vi "TrajectoryParam_enforceAccel.vi"(8 "TRAJECTORY_CONFIG":T1 {"End Velocity" format="%20.4f"; "StartVelocity" format="%20.4f"; "Max Acceleration" format="%20.4f"; "MaxVelocity" format="%20.4f"}, 10 "Reversed":bool, 11 "inCONSTRAINED_STATE":T2={"POSEwCURVATURE"={"CURVATURE"=0.0, "POSE"={"TRANSLATION"={"X"=0.0, "Y"=0.0}, "ROTATION"={"VALUE"=0.0, "COS"=1.0, "SIN"=0.0}}}, "Distance"=0.0, "minAccel"=0.0, "maxAccel"=0.0, "maxVelocity"=0.0} {"POSEwCURVATURE"."POSE"."ROTATION"."SIN" format="%13.4f"; "POSEwCURVATURE"."POSE"."ROTATION"."COS" format="%13.4f"; "POSEwCURVATURE"."POSE"."ROTATION"."VALUE" format="%13.4f"; "POSEwCURVATURE"."POSE"."TRANSLATION"."Y" format="%14.3f"; "POSEwCURVATURE"."POSE"."TRANSLATION"."X" format="%14.3f"}) -> (0 "error out":errorcluster, 3 "outCONSTRAINED_STATE":T2={"POSEwCURVATURE"={"CURVATURE"=0.0, "POSE"={"TRANSLATION"={"X"=0.0, "Y"=0.0}, "ROTATION"={"VALUE"=0.0, "COS"=1.0, "SIN"=0.0}}}, "Distance"=0.0, "minAccel"=0.0, "maxAccel"=0.0, "maxVelocity"=0.0} {"POSEwCURVATURE"."POSE"."ROTATION"."SIN" format="%13.4f"; "POSEwCURVATURE"."POSE"."ROTATION"."COS" format="%13.4f"; "POSEwCURVATURE"."POSE"."ROTATION"."VALUE" format="%13.4f"; "POSEwCURVATURE"."POSE"."TRANSLATION"."Y" format="%14.3f"; "POSEwCURVATURE"."POSE"."TRANSLATION"."X" format="%14.3f"})   [LabVIEW 2019, in "Trajectory_Library.lvlib"]
doc: "Internal routine called by TrajectoryParam_timeParam.VI \n\nThis routine enforces acceleration constraints and updates the ConstrainedState value based on the calculated limits.\n\nThis routine will need to be updated whenever a new constrained state type is added.\n------------------------------------------------------------------------------------------\n\nParameters:\n - InConstrainedState\n - Reversed\n - TrajectoryConfig\n\nReturns\n - OutConstrainedState"
uses:
  Trajectory_Library.lvlib
  <vilib>/Utility/Data Type/NI_Data Type.lvlib
  TypeDef/TRAJ_CONSTRAINT_CENTRIPETAL_ACCEL.ctl
  TypeDef/DIFF_DRIVE_KINEMATICS.ctl
  TypeDef/TRAJ_CONSTRAINT_DIIF_DRIVE_KINEMATICS.ctl
  TypeDef/SIMPLE_MOTOR_FF.ctl
  TypeDef/TRAJ_CONSTRAINT_DIIF_DRIVE_VOLTAGE.ctl
  TypeDef/TRANSLATION2D.ctl
  <vilib>/Analysis/Matrix/Datatypes/RealMatrix.ctl
  <vilib>/Analysis/Matrix/NI_Matrix.lvlib
  TypeDef/MECA_DRIVE_KINEMATICS.ctl
  TypeDef/TRAJ_CONSTRAINT_MECA_DRIVE_KINEMATICS.ctl
  TypeDef/SWERVE_DRIVE_KINEMATICS.ctl
  TypeDef/TRAJ_CONSTRAINT_SWERVE_DRIVE_KINEMATICS.ctl
  TypeDef/TRAJ_CONSTRAINT_MAX_VELOCITY.ctl
  Enum/TRAJ_CONSTRAINT_TYPES_ENUM.ctl
  TypeDef/TRAJ_CONSTRAINT_ELLIP_REGION.ctl
  TypeDef/TRAJ_CONSTRAINT_RECT_REGION.ctl
  TypeDef/ROTATION2D.ctl
  TypeDef/SWERVE_DRIVE_MODULE_STATE.ctl
  TypeDef/POSE2D.ctl
  TypeDef/POSEwCURVATURE.ctl
  TypeDef/CONSTRAINED_STATE.ctl
  TypeDef/TRAJ_CONFIG.ctl
panel:
  # "All units\nare SI"
  # "All units\nare SI"
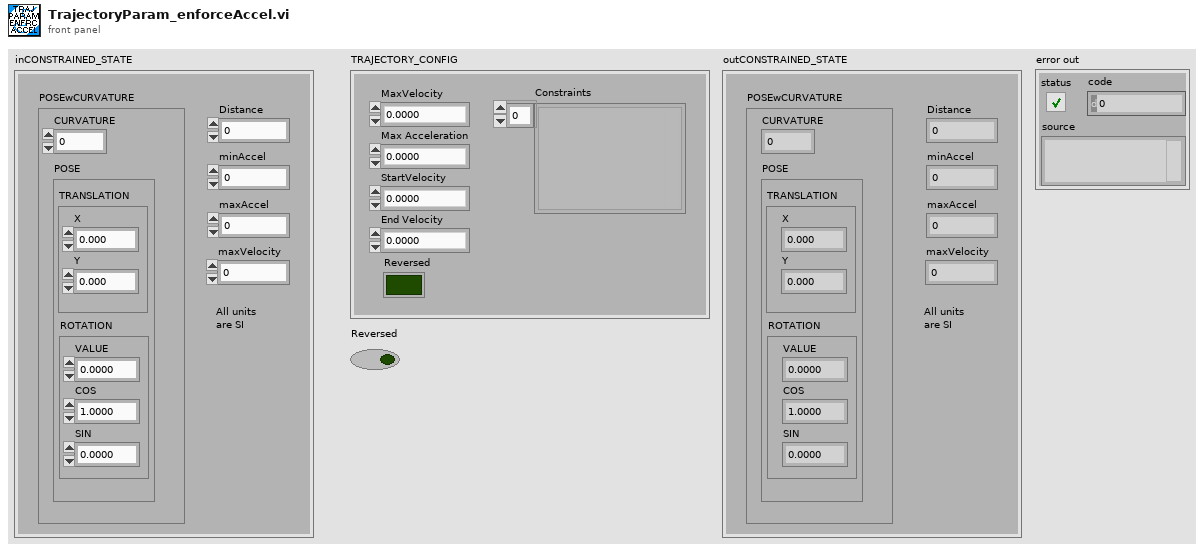
[diagram p1: front panel]
types:
  T1 = typedef "Trajectory_Library.lvlib/TRAJ_CONFIG.ctl" = cluster{"MaxVelocity":dbl, "Max Acceleration":dbl, "StartVelocity":dbl, "End Velocity":dbl, "Reversed":bool, "Constraints":variant[]}
  T2 = typedef "Trajectory_Library.lvlib/CONSTRAINED_STATE.ctl" = cluster{"POSEwCURVATURE":T3, "Distance":dbl, "minAccel":dbl, "maxAccel":dbl, "maxVelocity":dbl}
  T3 = typedef "Trajectory_Library.lvlib/POSEwCURVATURE.ctl" = cluster{"CURVATURE":dbl, "POSE":T4}
  T4 = typedef "Trajectory_Library.lvlib/POSE2D.ctl" = cluster{"TRANSLATION":T5, "ROTATION":T6}
  T5 = typedef "Trajectory_Library.lvlib/TRANSLATION2D.ctl" = cluster{"X":dbl, "Y":dbl}
  T6 = typedef "Trajectory_Library.lvlib/ROTATION2D.ctl" = cluster{"VALUE":dbl, "COS":dbl, "SIN":dbl}
  T7 = typedef "Trajectory_Library.lvlib/TRAJ_CONSTRAINT_DIIF_DRIVE_KINEMATICS.ctl" = cluster{"Max Speed (M/S)":dbl, "DIFF_DRIVE_KINEMATICS":T8, "Max Accel (M/S2)":dbl}
  T8 = typedef "Trajectory_Library.lvlib/DIFF_DRIVE_KINEMATICS.ctl" = cluster{"TrackWidth_Meters":dbl}
  T9 = typedef "Trajectory_Library.lvlib/TRAJ_CONSTRAINT_CENTRIPETAL_ACCEL.ctl" = cluster{"Max Cent Accel":dbl}
  T10 = typedef "Trajectory_Library.lvlib/TRAJ_CONSTRAINT_DIIF_DRIVE_VOLTAGE.ctl" = cluster{"Max Voltage":dbl, "DIFF_DRIVE_KINEMATICS":T8, "SIMPLE_MOTOR_FF":T11}
  T11 = typedef "Trajectory_Library.lvlib/SIMPLE_MOTOR_FF.ctl" = cluster{"Ks":dbl, "Kv":dbl, "Ka":dbl, "KnInv":dbl}
  T12 = typedef "Trajectory_Library.lvlib/TRAJ_CONSTRAINT_MECA_DRIVE_KINEMATICS.ctl" = cluster{"Max Speed (M/S)":dbl, "MECA_DRIVE_KINEMATICS":T13}
  T13 = typedef "Trajectory_Library.lvlib/MECA_DRIVE_KINEMATICS.ctl" = cluster{"FrontLeft":T5, "FrontRight":T5, "RearLeft":T5, "RearRight":T5, "InverseKinematics":T14, "ForwardKinematics":T14, "PrevCoR":T5}
  T14 = typedef "NI_Matrix.lvlib/RealMatrix.ctl" = dbl[][]
  T15 = typedef "Trajectory_Library.lvlib/TRAJ_CONSTRAINT_SWERVE_DRIVE_KINEMATICS.ctl" = cluster{"Max Speed (M/S)":dbl, "SwerveKinematics":T16}
  T16 = typedef "Trajectory_Library.lvlib/SWERVE_DRIVE_KINEMATICS.ctl" = cluster{"NumModules":i32, "InverseKinematics":T14, "ForwardKinematics":T14, "Modules":T5[], "PrevCoR":T5, "SavedModuleStates":T17[]}
  T17 = typedef "Trajectory_Library.lvlib/SWERVE_DRIVE_MODULE_STATE.ctl" = cluster{"Speed":dbl, "Angle":T6}
  T18 = typedef "Trajectory_Library.lvlib/TRAJ_CONSTRAINT_MAX_VELOCITY.ctl" = cluster{"Max Velocity":dbl, "IM UNIQUE":bool}
  T19 = typedef "Trajectory_Library.lvlib/TRAJ_CONSTRAINT_ELLIP_REGION.ctl" = cluster{"Center":T5, "Radii":T5, "Constraint":variant, "Constraint Type":T20, "IM UNIQUE":bool}
  T20 = typedef "Trajectory_Library.lvlib/TRAJ_CONSTRAINT_TYPES_ENUM.ctl" = enum16{"UNDEFINED", "DIFF DRIVE KINEMATICS", "DIFF DRIVE VOLTAGE", "CENTRIPITAL ACCEL", "MECA DRIVE KINEMATICS", "SWERVE DRIVE KINEMATICS", "MAXIMUM VELOCITY", "ELLIPTICAL REGION", "RECTANGULAR REGION"}
  T21 = typedef "Trajectory_Library.lvlib/TRAJ_CONSTRAINT_RECT_REGION.ctl" = cluster{"BottomLeftPoint":T5, "TopRightPoint":T5, "Constraint":variant, "Constraint Type":T20}
  T22 = typedef "Trajectory_Library.lvlib/TRAJ_CONSTRAINT_MINMAX.ctl" = cluster{"minAccel":dbl, "maxAccel":dbl}
  T23 = typedef "WPILib_Math.lvlib/TRAJ_CONSTRAINT_MINMAX.ctl" = cluster{"minAccel":dbl, "maxAccel":dbl}
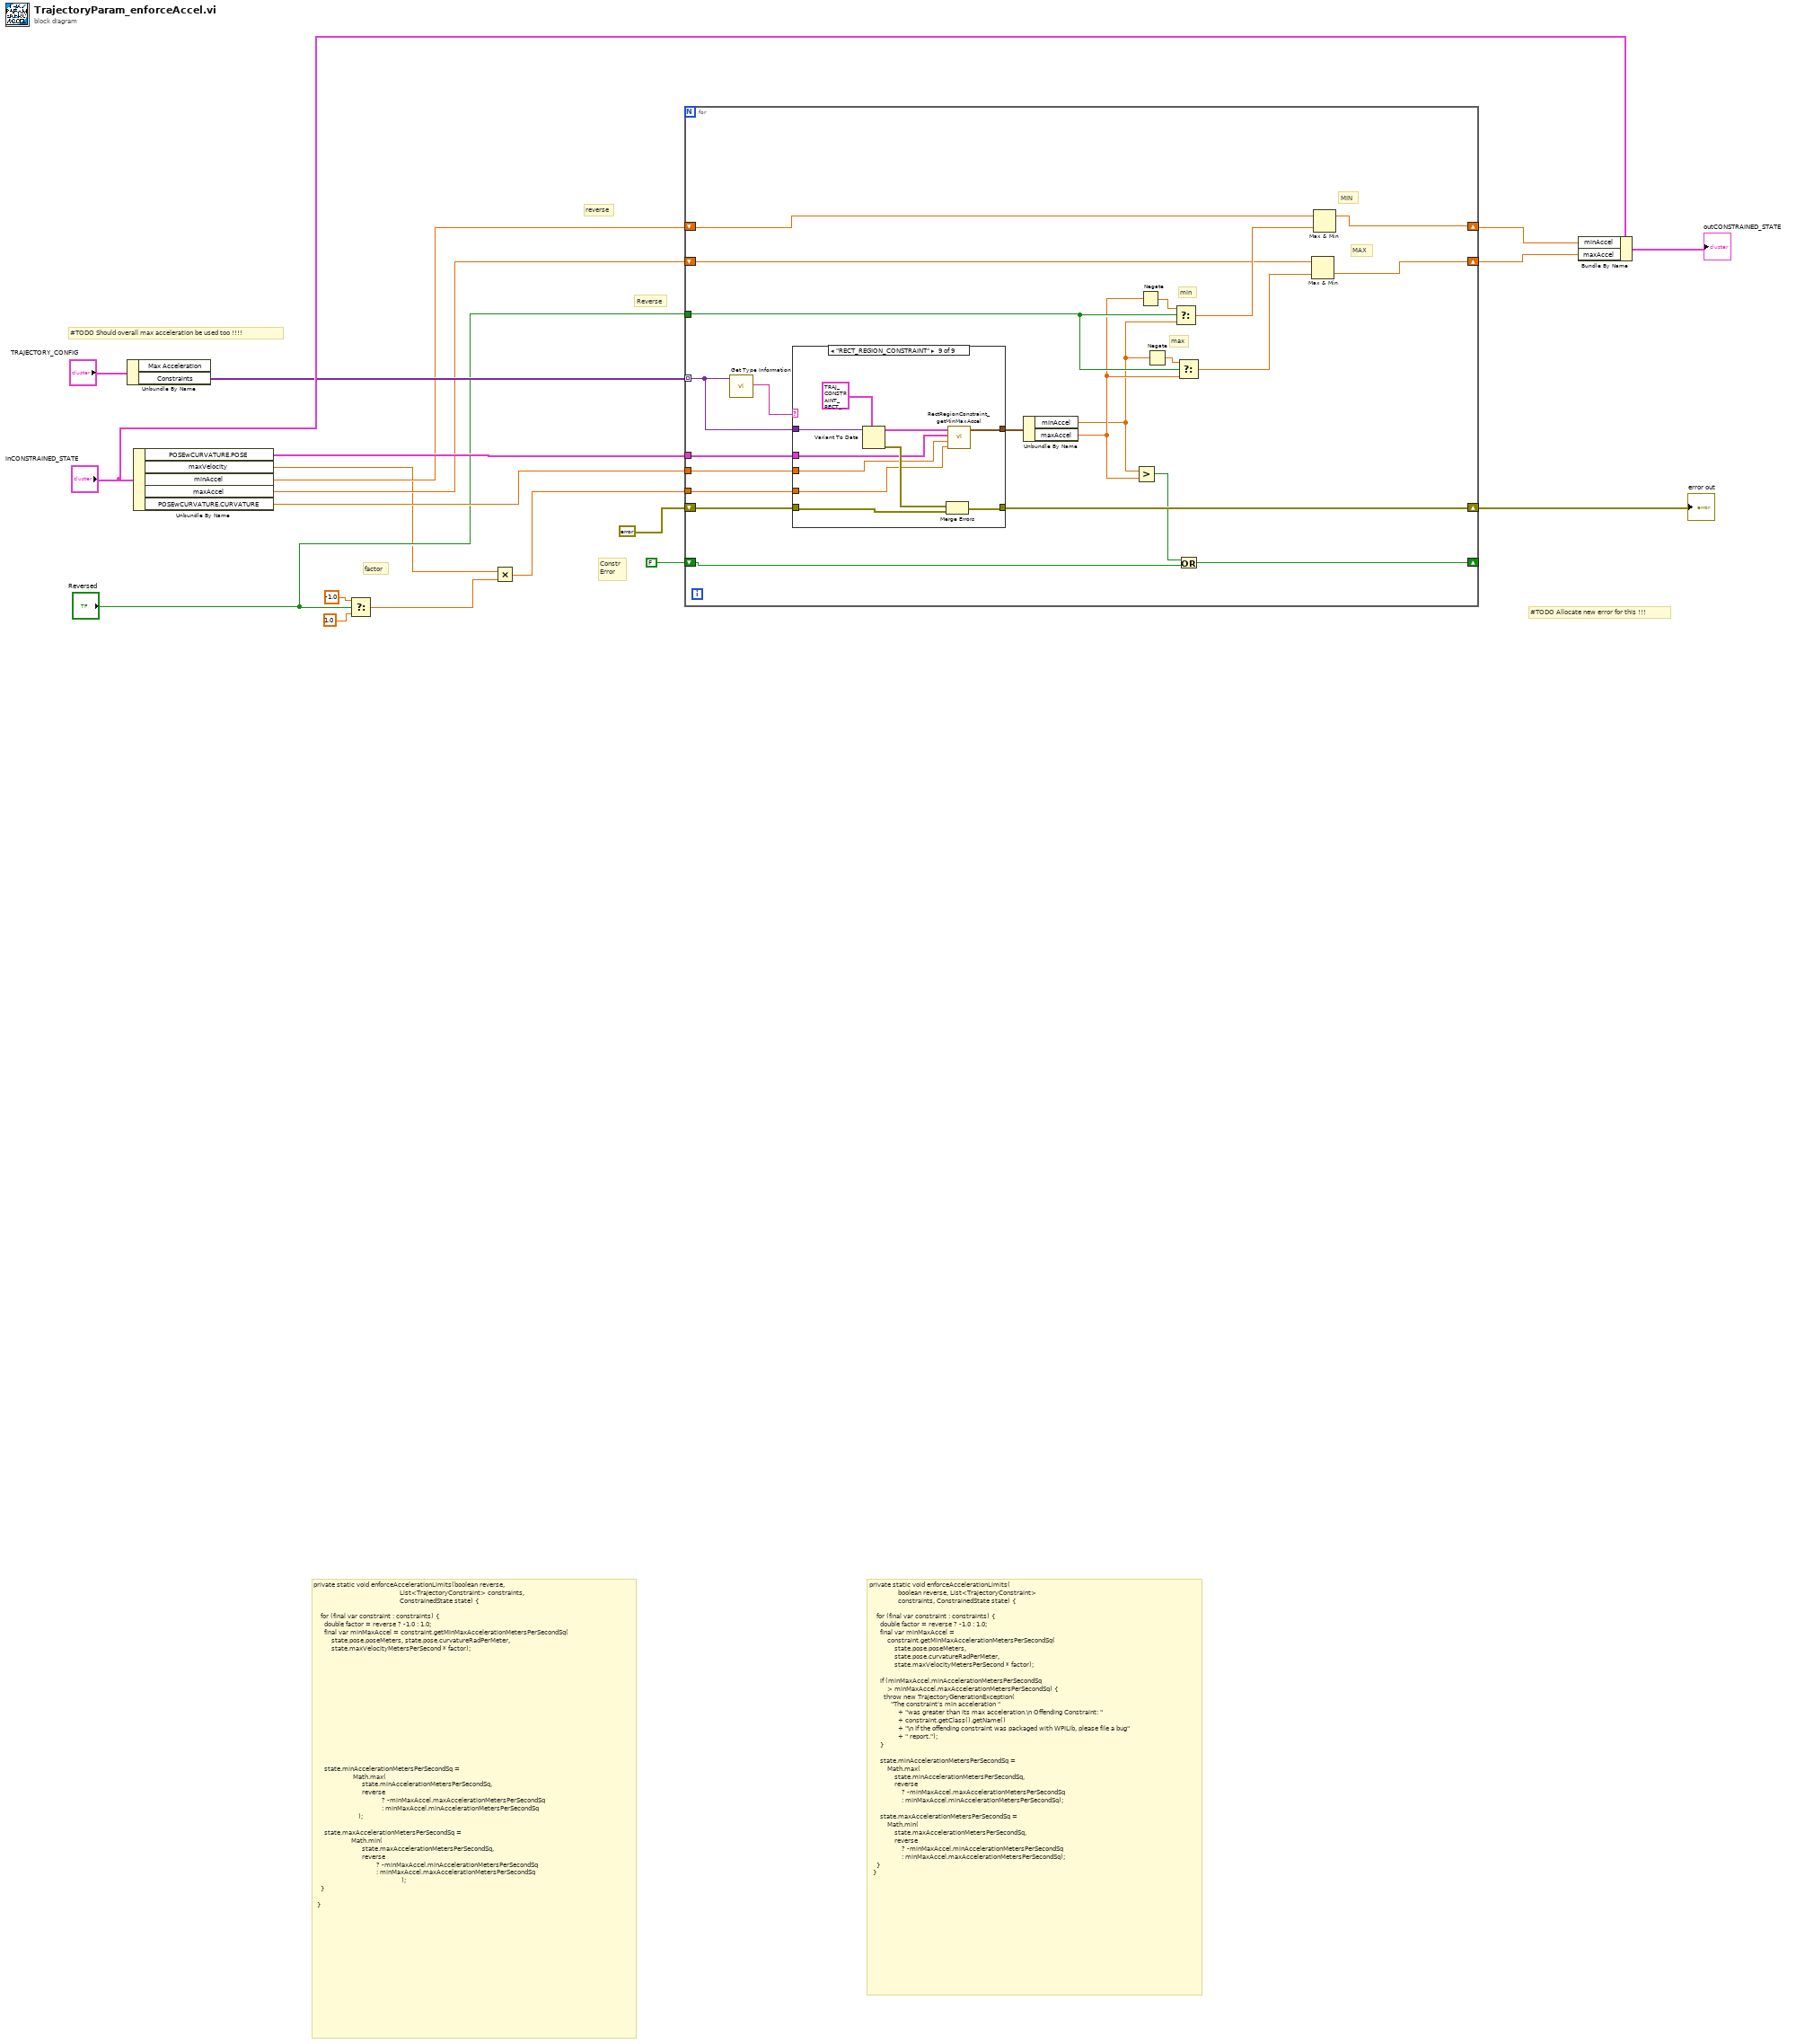
[diagram p0: block diagram]
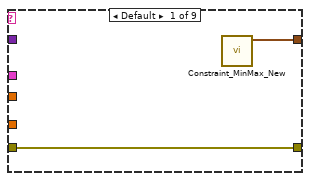
[diagram p2: hidden frame]
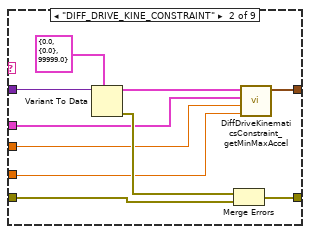
[diagram p3: hidden frame]
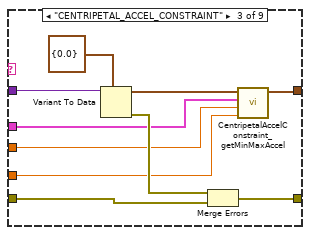
[diagram p4: hidden frame]
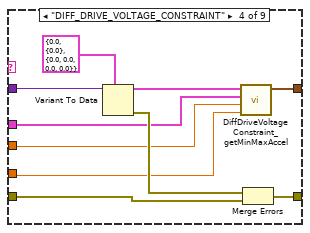
[diagram p5: hidden frame]
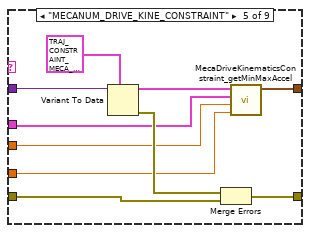
[diagram p6: hidden frame]
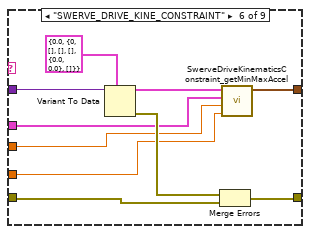
[diagram p7: hidden frame]
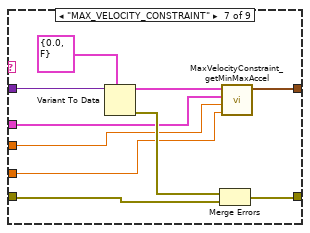
[diagram p8: hidden frame]
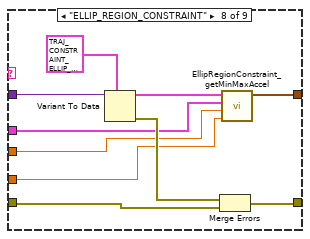
[diagram p9: hidden frame]
diagram:
  # "#TODO Allocate new error for this !!!"
  # "#TODO Should overall max acceleration be used too !!!!"
  # "Reverse"
  # "reverse"
  # "Constr\nError"
  # "private static void enforceAccelerationLimits(\n                boolean reverse, List<TrajectoryConstraint> \n                constraints, ConstrainedState state) {\n\n    for (final var constraint : constraints) {\n      double factor = reverse ? -1.0 : 1.0;\n      final var minMaxAccel =\n          constraint.getMinMaxAccelerationMetersPerSecondSq(\n              state.pose.poseMeters,\n              state.pose.curvatureRadPerMeter,\n              state.maxVelocityMetersPerSecond * factor);\n\n      if (minMaxAccel.minAccelerationMetersPerSecondSq\n          > minMaxAccel.maxAccelerationMetersPerSecondSq) {\n        throw new TrajectoryGenerationException(\n            \"The constraint's min acceleration \"\n                + \"was greater than its max acceleration.\\n Offending Constraint: \"\n                + constraint.getClass().getName()\n                + \"\\n If the offending constraint was packaged with WPILib, please file a bug\"\n                + \" report.\");\n      }\n\n      state.minAccelerationMetersPerSecondSq =\n          Math.max(\n              state.minAccelerationMetersPerSecondSq,\n              reverse\n                  ? -minMaxAccel.maxAccelerationMetersPerSecondSq\n                  : minMaxAccel.minAccelerationMetersPerSecondSq);\n\n      state.maxAccelerationMetersPerSecondSq =\n          Math.min(\n              state.maxAccelerationMetersPerSecondSq,\n              reverse\n                  ? -minMaxAccel.minAccelerationMetersPerSecondSq\n                  : minMaxAccel.maxAccelerationMetersPerSecondSq);\n    }\n  }"
  # "factor"
  # "private static void enforceAccelerationLimits(boolean reverse,\n                                                List<TrajectoryConstraint> constraints,\n                                                ConstrainedState state) {\n\n    for (final var constraint : constraints) {\n      double factor = reverse ? -1.0 : 1.0;\n      final var minMaxAccel = constraint.getMinMaxAccelerationMetersPerSecondSq(\n          state.pose.poseMeters, state.pose.curvatureRadPerMeter,\n          state.maxVelocityMetersPerSecond * factor);\n\n\n\n\n\n\n\n\n\n\n\n\n\n\n      state.minAccelerationMetersPerSecondSq = \n                      Math.max(\n                           state.minAccelerationMetersPerSecondSq,\n                           reverse \n                                      ? -minMaxAccel.maxAccelerationMetersPerSecondSq \n                                      : minMaxAccel.minAccelerationMetersPerSecondSq\n                         );\n\n      state.maxAccelerationMetersPerSecondSq = \n                     Math.min(\n                           state.maxAccelerationMetersPerSecondSq,\n                           reverse \n                                   ? -minMaxAccel.minAccelerationMetersPerSecondSq \n                                   : minMaxAccel.maxAccelerationMetersPerSecondSq\n                                                 );\n    }\n\n  }"
  n1 = Unbundle By Name("TRAJECTORY_CONFIG") -> ("Constraints"=w14:variant[])  [unwired: 1 out]
  n2 = Unbundle By Name("inCONSTRAINED_STATE") -> ("POSEwCURVATURE.POSE"=w12:T4, "maxVelocity"=w2:dbl, "minAccel"=w6:dbl, "maxAccel"=w7:dbl, "POSEwCURVATURE.CURVATURE"=w11:dbl)
  n3 = Select(t=-1.0, s="Reversed", f=1.0) -> (s? t:f=w1:dbl)
  n4 = Multiply(x=w2, y=w1) -> (x*y=w10:dbl)
  n5 = for {
    tunnel: w14 -> [w40] mode=indexing
    tunnel: w12 -> [w39]
    tunnel: w11 -> [w38]
    tunnel: w10 -> [w37]
    shift-right: [w36] -> w5
    shift-left: errorcluster {"status"=FALSE, "code"=0, "source"=""} ("error IO") -> [w35]
    shift-right: [w32] -> _
    shift-left: FALSE -> [w31]
    tunnel: "Reversed" -> [w30]
    shift-right: [w22] -> w4
    shift-left: w6 -> [w27]
    shift-right: [w21] -> w3
    shift-left: w7 -> [w25]
    # "MAX"
    # "MIN"
    # "max"
    # "min"
    n6 = call <vilib>:"Get Type Information.vi"("variant"=w40) -> ("name"=w41:string)  [unwired: 6 in, 4 out]
    n7 = case shown="\"RECT_REGION_CONSTRAINT\"" w41 {
      tunnel: w40 -> [_ w53 w63 w73 w83 w93 w103 w113 w123]
      tunnel: w39 -> [_ w46 w56 w66 w76 w87 w97 w107 w117]
      tunnel: w38 -> [_ w45 w55 w65 w75 w86 w96 w106 w116]
      tunnel: w37 -> [_ w44 w54 w64 w74 w85 w95 w105 w115]
      tunnel: [w43 w51 w62 w71 w82 w92 w102 w112 w122] -> w36
      tunnel: w35 -> [w43 w50 w60 w70 w80 w90 w100 w110 w120]
      tunnel: [w42 w48 w58 w68 w78 w84 w94 w104 w114] -> w34
      frame Default {
        n8 = call "Constraint_MinMax_New.vi"() -> ("TRAJ_CONSTAINT_MIN_MAX"=w42:T22)  [unwired: 11 in]
      }
      frame "DIFF_DRIVE_KINE_CONSTRAINT" {
        n9 = Variant To Data(type=T7 {"Max Speed (M/S)"=0.0, "DIFF_DRIVE_KINEMATICS"={"TrackWidth_Meters"=0.0}, "Max Accel (M/S2)"=99999.0} ("DIFF_DRIVE_KINE_CONSTRAINT"), Variant=w53) -> (data=w47:T7, error out=w52:errorcluster)  [unwired: 1 in]
        n10 = Merge Errors(w52, w50) -> (w51:errorcluster)
        n11 = call "DiffDriveKinematicsConstraint_getMinMaxAccel.vi"("Velocity_M/S"=w44, "Curvature"=w45, "statePose"=w46, "DIFF_DRIVE_KINE_CONSTRAINT"=w47) -> ("TRAJ_CONSTAINT_MIN_MAX"=w48:T23)  [unwired: 7 in]
      }
      frame "CENTRIPETAL_ACCEL_CONSTRAINT" {
        n12 = Variant To Data(type=T9 {"Max Cent Accel"=0.0} ("CENTRIPETAL_ACCEL_CONSTRAINT"), Variant=w63) -> (data=w57:T9, error out=w61:errorcluster)  [unwired: 1 in]
        n13 = Merge Errors(w61, w60) -> (w62:errorcluster)
        n14 = call "CentripetalAccelConstraint_getMinMaxAccel.vi"("maxVelocity"=w54, "Curvature"=w55, "statePose"=w56, "CENTRIPETAL_ACCEL_CONSTRAINT"=w57) -> ("TRAJ_CONSTAINT_MIN_MAX"=w58:T23)  [unwired: 7 in]
      }
      frame "DIFF_DRIVE_VOLTAGE_CONSTRAINT" {
        n15 = Variant To Data(type=T10 {"Max Voltage"=0.0, "DIFF_DRIVE_KINEMATICS"={"TrackWidth_Meters"=0.0}, "SIMPLE_MOTOR_FF"={"Ks"=0.0, "Kv"=0.0, "Ka"=0.0, "KnInv"=0.0}} ("DIFF_DRIVE_VOLTAGE_CONSTRAINT"), Variant=w73) -> (data=w67:T10, error out=w72:errorcluster)  [unwired: 1 in]
        n16 = call "DiffDriveVoltageConstraint_getMinMaxAccel.vi"("Velocity"=w64, "Curvature"=w65, "statePose"=w66, "DIFF_DRIVE_VOLTAGE_CONSTRAINT"=w67) -> ("TRAJ_CONSTAINT_MIN_MAX"=w68:T22)  [unwired: 7 in]
        n17 = Merge Errors(w72, w70) -> (w71:errorcluster)
      }
      frame "MECANUM_DRIVE_KINE_CONSTRAINT" {
        n18 = Variant To Data(type=T12 {"Max Speed (M/S)"=0.0, "MECA_DRIVE_KINEMATICS"={"FrontLeft"={"X"=0.0, "Y"=0.0}, "FrontRight"={"X"=0.0, "Y"=0.0}, "RearLeft"={"X"=0.0, "Y"=0.0}, "RearRight"={"X"=0.0, "Y"=0.0}, "InverseKinematics"=[[0.0, 1.0, -1.0, 0.0], [0.0, 1.0, 1.0, 0.0], [0.0, 1.0, 1.0, 0.0], [0.0, 1.0, -1.0, 0.0]], "ForwardKinematics"=[[0.0, 1.0, -1.0, 0.0], [0.0, 1.0, 1.0, 0.0], [0.0, 1.0, 1.0, 0.0], [0.0, 1.0, -1.0, 0.0]], "PrevCoR"={"X"=0.0, "Y"=0.0}}} ("MECANUM_DRIVE_KINE_CONSTRAINT"), Variant=w83) -> (data=w77:T12, error out=w81:errorcluster)  [unwired: 1 in]
        n19 = Merge Errors(w81, w80) -> (w82:errorcluster)
        n20 = call "MecaDriveKinematicsConstraint_getMinMaxAccel.vi"("maxVelocity"=w74, "Curvature"=w75, "statePose"=w76, "MECANUM_DRIVE_KINE_CONSTRAINT"=w77) -> ("TRAJ_CONSTAINT_MIN_MAX"=w78:T23)  [unwired: 7 in]
      }
      frame "SWERVE_DRIVE_KINE_CONSTRAINT" {
        n21 = Variant To Data(type=T15 {"Max Speed (M/S)"=0.0, "SwerveKinematics"={"NumModules"=0, "InverseKinematics"=[], "ForwardKinematics"=[], "Modules"=[], "PrevCoR"={"X"=0.0, "Y"=0.0}, "SavedModuleStates"=[]}} ("SWERVE_DRIVE_KINE_CONSTRAINT"), Variant=w93) -> (data=w88:T15, error out=w91:errorcluster)  [unwired: 1 in]
        n22 = Merge Errors(w91, w90) -> (w92:errorcluster)
        n23 = call "SwerveDriveKinematicsConstraint_getMinMaxAccel.vi"("maxVelocity"=w85, "Curvature"=w86, "statePose"=w87, "SWERVE_DRIVE_KINE_CONSTRAINT"=w88) -> ("TRAJ_CONSTAINT_MIN_MAX"=w84:T22)  [unwired: 7 in]
      }
      frame "MAX_VELOCITY_CONSTRAINT" {
        n24 = Variant To Data(type=T18 {"Max Velocity"=0.0, "IM UNIQUE"=FALSE} ("MAX_VELOCITY_CONSTRAINT"), Variant=w103) -> (data=w98:T18, error out=w101:errorcluster)  [unwired: 1 in]
        n25 = Merge Errors(w101, w100) -> (w102:errorcluster)
        n26 = call "MaxVelocityConstraint_getMinMaxAccel.vi"("maxVelocity"=w95, "Curvature"=w96, "statePose"=w97, "MAX_VELOCITY_CONSTRAINT"=w98) -> ("TRAJ_CONSTAINT_MIN_MAX"=w94:T22)  [unwired: 7 in]
      }
      frame "ELLIP_REGION_CONSTRAINT" {
        n27 = Variant To Data(type=T19 {"Center"={"X"=0.0, "Y"=0.0}, "Radii"={"X"=0.0, "Y"=0.0}, "Constraint"=variant, "Constraint Type"=enum."DIFF DRIVE KINEMATICS", "IM UNIQUE"=FALSE} ("ELLIP_REGION_CONSTRAINT"), Variant=w113) -> (data=w108:T19, error out=w111:errorcluster)  [unwired: 1 in]
        n28 = Merge Errors(w111, w110) -> (w112:errorcluster)
        n29 = call "EllipRegionConstraint_getMinMaxAccel.vi"("Velocity_M/S"=w105, "Curvature"=w106, "statePose"=w107, "ELLIP REGION CONSTRAINT"=w108) -> ("TRAJ_CONSTAINT_MIN_MAX"=w104:T22)  [unwired: 7 in]
      }
      frame "RECT_REGION_CONSTRAINT" {
        n30 = Variant To Data(type=T21 {"BottomLeftPoint"={"X"=0.0, "Y"=0.0}, "TopRightPoint"={"X"=0.0, "Y"=0.0}, "Constraint"=variant, "Constraint Type"=enum."DIFF DRIVE KINEMATICS"} ("RECT_REGION_CONSTRAINT"), Variant=w123) -> (data=w118:T21, error out=w121:errorcluster)  [unwired: 1 in]
        n31 = Merge Errors(w121, w120) -> (w122:errorcluster)
        n32 = call "RectRegionConstraint_getMinMaxAccel.vi"("Velocity_M/S"=w115, "Curvature"=w116, "statePose"=w117, "RECT REGION CONSTRAINT"=w118) -> ("TRAJ_CONSTAINT_MIN_MAX"=w114:T23)  [unwired: 7 in]
      }
    }
    n33 = Unbundle By Name(w34) -> ("minAccel"=w20:dbl, "maxAccel"=w23:dbl)
    n34 = Greater?(x=w20, y=w23) -> (0:w33:bool)
    n35 = Negate(x=w23) -> (-x=w28:dbl)
    n36 = Negate(x=w20) -> (-x=w29:dbl)
    n37 = Select(t=w28, s=w30, f=w20) -> (s? t:f=w26:dbl)
    n38 = Select(t=w29, s=w30, f=w23) -> (s? t:f=w24:dbl)
    n39 = Or(x=w33, y=w31) -> (x .or. y?=w32:bool)
    n40 = Max & Min(x=w25, y=w24) -> (min(x,y)=w21:dbl)  [unwired: 1 out]
    n41 = Max & Min(x=w27, y=w26) -> (max(x,y)=w22:dbl)  [unwired: 1 out]
  }
  "error out" <- w5
  n42 = Bundle By Name(cluster="inCONSTRAINED_STATE", "minAccel"=w4, "maxAccel"=w3) -> (→"outCONSTRAINED_STATE":T2)
